vi "to string.vi"(8 "error in":errorcluster, 11 "configuration in":refnum<class "PL_Target Configuration.lvclass">=refnum) -> (0 "error out":errorcluster, 1 "data":string, 2 "version":string, 3 "configuration out":refnum<class "PL_Target Configuration.lvclass">)   [LabVIEW 2014, in "PL_Target Configuration.lvclass"]
doc: "Provides an interface for saving a module configuration to a file or other serialized data source. It is recommended that all children of this class store data in two sets--data required for its own initialization, and any data required for parent initialization--and that each implementation uses the <b>Call Parent Method</b> primitive to serialize parent information."
uses:
  PL_Target Configuration.lvclass
  <vilib>/NI/Configuration Framework/serializable configuration/NISE_CEF_serializable configuration.lvclass
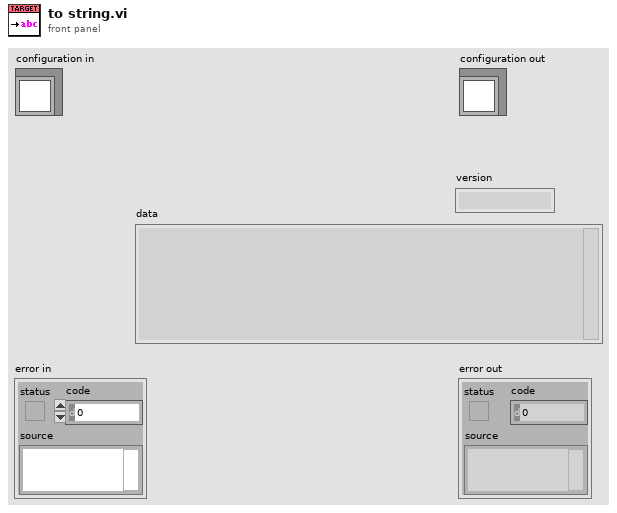
[diagram p1: front panel]
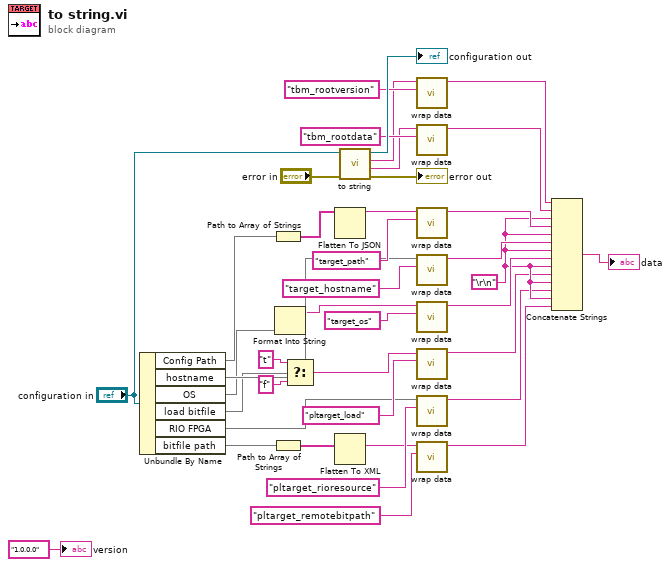
[diagram p0: block diagram]
diagram:
  w15 = "\r\n"
  n1 = Unbundle By Name("configuration in") -> ("Config Path"=w30, "hostname"=w22, "OS"=w19, "load bitfile"=w7, "RIO FPGA"=w8, "bitfile path"=w3)
  n2 = Path to Array of Strings(0:w30) -> (2:w29:string[])  [unwired: 1 out]
  n3 = Path to Array of Strings(0:w3) -> (2:w2:string[])  [unwired: 1 out]
  n4 = Format Into String(w19) -> (resulting string=w17:string)  [unwired: 3 in, 1 out]
  n5 = Select(t="t" ("additional identifier"), s=w7, f="f" ("additional identifier")) -> (s? t:f=w5:string)
  n6 = Flatten To JSON(anything=w29) -> (JSON string=w28:string)  [unwired: 2 in, 1 out]
  n7 = Flatten To XML(anything=w2) -> (xml string=w1:string)
  n8 = call-parent "to string.vi"("error in"="error in", "configuration in"="configuration in") -> ("error out"=→"error out":errorcluster, "data"=w32:string, "version"=w33:string, "configuration out"=→"configuration out":refnum<class "PL_Target Configuration.lvclass">)  [unwired: 6 in]
  n9 = call <vilib>:"wrap data.vi"("identifier"="tbm_rootversion" ("additional identifier"), "data to wrap"=w33) -> ("wrapped data"=w27:string)  [unwired: 9 in]
  n10 = call <vilib>:"wrap data.vi"("identifier"="tbm_rootdata" ("additional identifier"), "data to wrap"=w32) -> ("wrapped data"=w26:string)  [unwired: 9 in]
  n11 = call <vilib>:"wrap data.vi"("identifier"="target_path" ("additional identifier"), "data to wrap"=w28) -> ("wrapped data"=w25:string)  [unwired: 9 in]
  n12 = call <vilib>:"wrap data.vi"("identifier"="target_hostname" ("additional identifier"), "data to wrap"=w22) -> ("wrapped data"=w20:string)  [unwired: 9 in]
  n13 = call <vilib>:"wrap data.vi"("identifier"="target_os" ("additional identifier"), "data to wrap"=w17) -> ("wrapped data"=w16:string)  [unwired: 9 in]
  n14 = call <vilib>:"wrap data.vi"("identifier"="pltarget_load" ("additional identifier"), "data to wrap"=w5) -> ("wrapped data"=w14:string)  [unwired: 9 in]
  n15 = call <vilib>:"wrap data.vi"("identifier"="pltarget_rioresource" ("additional identifier"), "data to wrap"=w8) -> ("wrapped data"=w13:string)  [unwired: 9 in]
  n16 = call <vilib>:"wrap data.vi"("identifier"="pltarget_remotebitpath" ("additional identifier"), "data to wrap"=w1) -> ("wrapped data"=w12:string)  [unwired: 9 in]
  n17 = Concatenate Strings(w27, w26, w15, w25, w15, w20, w15, w16, w15, w14, w15, w13, w15, w12) -> (→"data":string)
  "version" <- "1.0.0.0" ("version")
